vi "Enqueue Message (Array).vi"(6 "Priority Message? Array":bool[](array[boolean]), 8 "error in (no error)":errorcluster, 9 "Message Data Array":variant[](array[variant]), 10 "Array":T1[](array[typedef]), 11 "Message Queue":refnum<queue>) -> (0 "error out":errorcluster, 3 "dup Message Queue":refnum<queue>)   [LabVIEW 2021, in "Message Queue.lvlib"]
doc: "For a regular message, enqueue the message. For a priority message, enqueue it at the front of the queue."
uses:
  Message Queue.lvlib
  Message Cluster.ctl
  controls/test_sequence .ctl
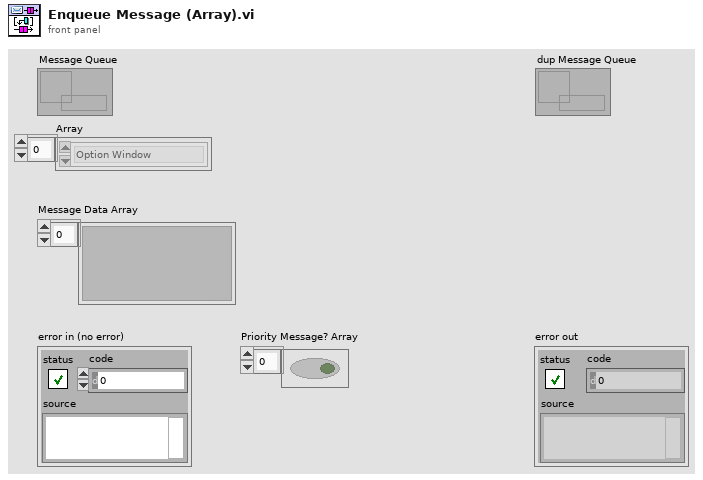
[diagram p1: front panel]
types:
  T1 = typedef "test_sequence .ctl" = enum16{"Init Devices", "Login", "Option Window", "Idle state", "Check", "Uncheck", "Scan Barcode", "Clear the test Containers", "Init-Pre Test", "Test ", "Result", "Report", "Database", "Update Display", "Confirm Quit", "Error", "Exit"}
  T2 = typedef "Message Queue.lvlib/Message Cluster.ctl" = cluster{"Message":T1, "Message Data":variant}
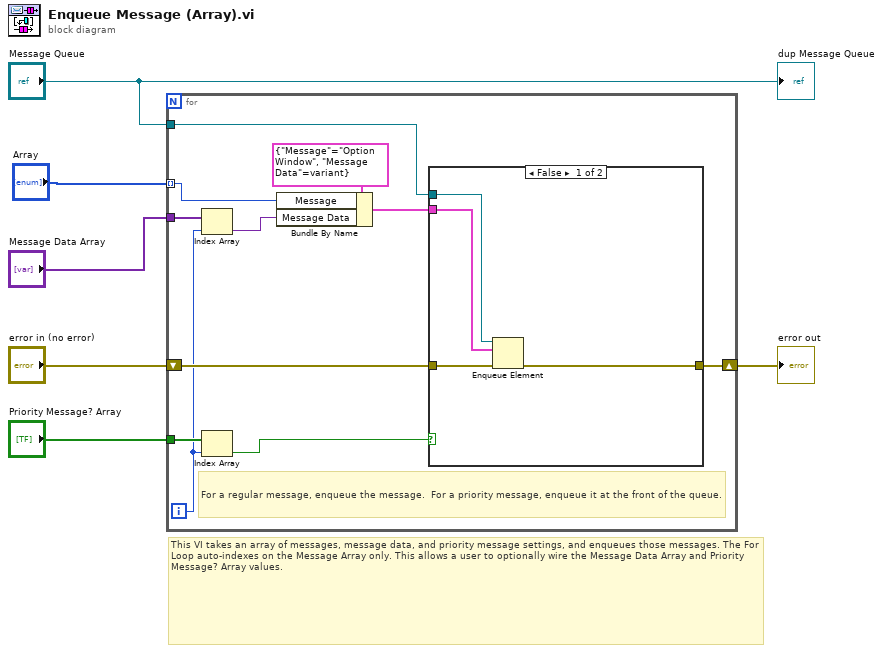
[diagram p0: block diagram]
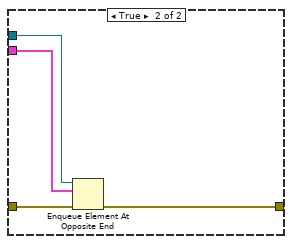
[diagram p2: hidden frame]
diagram:
  # "This VI takes an array of messages, message data, and priority message settings, and enqueues those messages. The For Loop auto-indexes on the Message Array only. This allows a user to optionally wire the Message Data Array and Priority Message? Array values."
  n1 = for {
    tunnel: "Message Data Array" -> [w12]
    tunnel: "Priority Message? Array" -> [w10]
    tunnel: "Message Queue" -> [w14]
    shift-right: [w15] -> w3
    shift-left: "error in (no error)" -> [w16]
    tunnel: "Array" -> [w7] mode=indexing
    i -> [w8]
    # "For a regular message, enqueue the message.  For a priority message, enqueue it at the front of the queue."
    n2 = Index Array(array=w12, index=w8) -> (element=w11:variant)
    n3 = Index Array(array=w10, index=w8) -> (element=w9:bool)
    n4 = Bundle By Name(cluster=T2 {"Message"=enum."Option Window", "Message Data"=variant} ("Message Cluster"), "Message"=w7, "Message Data"=w11) -> (w13:T2)
    n5 = case shown="False" w9 {
      tunnel: w16 -> [w21 w25]
      tunnel: [w20 w24] -> w15
      tunnel: w14 -> [w19 w23]
      tunnel: w13 -> [w18 w22]
      frame False {
        n6 = Enqueue Element(queue=w19, element=w18, error in (no error)=w21) -> (error out=w20:errorcluster)  [unwired: 1 in, 2 out]
      }
      frame True {
        n7 = Enqueue Element At Opposite End(queue=w23, element=w22, error in (no error)=w25) -> (error out=w24:errorcluster)  [unwired: 1 in, 2 out]
      }
    }
  }
  "error out" <- w3
  "dup Message Queue" <- "Message Queue"
